vi "Render_AD_Results.vi"(4 "Background Color":u32(colorbox)=16448250, 5 "Rel._Margin":sgl=0.01, 8 "error in":errorcluster, 11 "Anomaly Detection Rresults":T1={"Image"="remote image 000001443E0F18B8", "Ground Truth"="remote image 000001443E0F3018", "Predicted Heat Map"="remote image 000001443E0F25C8", "Predicted Mask"="remote image 000001443E0F1808", "Segmentation"="remote image 000001443E0F2E08"}) -> (0 "error out":errorcluster, 3 "Anomaly Detection Result":T2(plugin-control))   [LabVIEW 2020]
uses:
  Controls/Anomaly_Detection_Results_Imgs.ctl
  <vilib>/vision/NI_Vision_Development_Module.lvlib
panel:
  out "Font Size 2":i16
  in  "Desired Font (Application)":T3(ring)
  in  "[User-specified Font].Font Name":string="system font"
  in  "Horizontal Alignment":i16(ring)=1 items=["Left", "Center", "Right"]
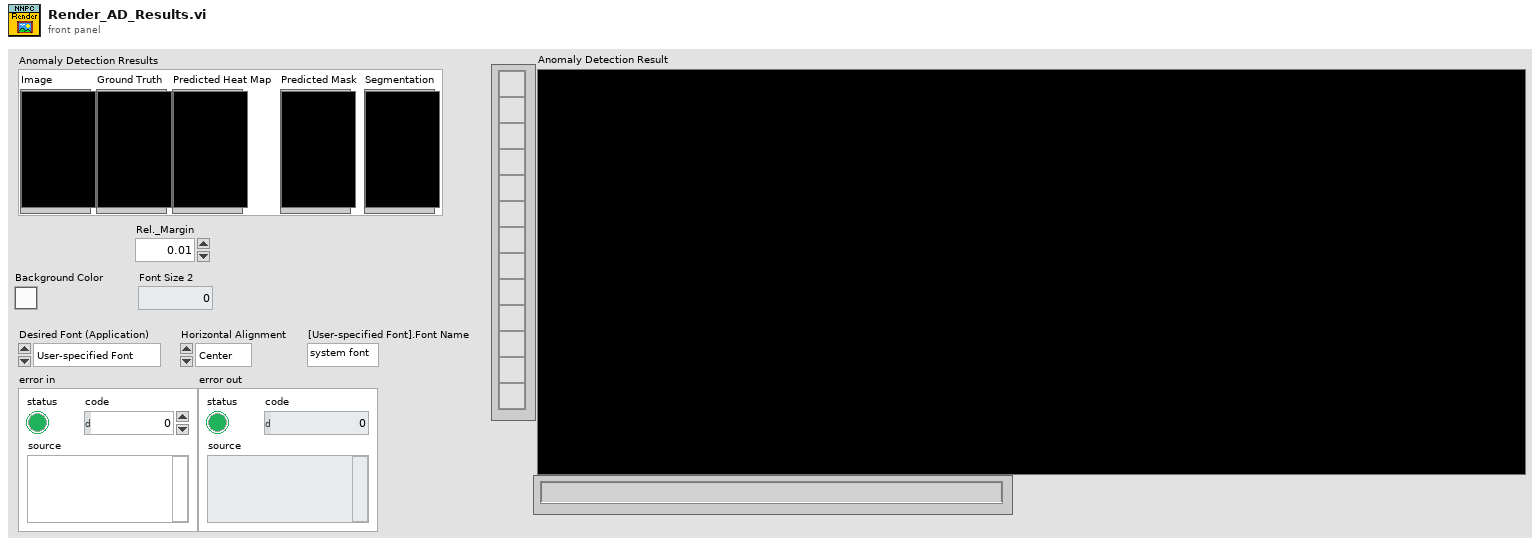
[diagram p1: front panel]
types:
  T1 = typedef "Anomaly_Detection_Results_Imgs.ctl" = cluster{"Image":T2, "Ground Truth":T2, "Predicted Heat Map":T2, "Predicted Mask":T2, "Segmentation":T2}
  T2 = typedef "IMAQ Image.ctl" = refnum<image>
  T3 = enum16{"User-specified Font", "Application Font", "System Font", "Dialog Font"}
  T4 = cluster{"Desired Font (Application)":enum16{"User-specified Font", "Application Font", "System Font", "Dialog Font"}, "[User-specified Font]":cluster{"Font Name":string, "Size":i16, "Strikeout?":bool, "Italic?":bool, "Underline?":bool, "Outline?":bool, "Shadow?":bool, "Bold?":bool, "Rotation Angle":dbl}, "Horizontal Alignment":i16, "Vertical Alignment":i16}
  T5 = typedef "Image Type" = u32
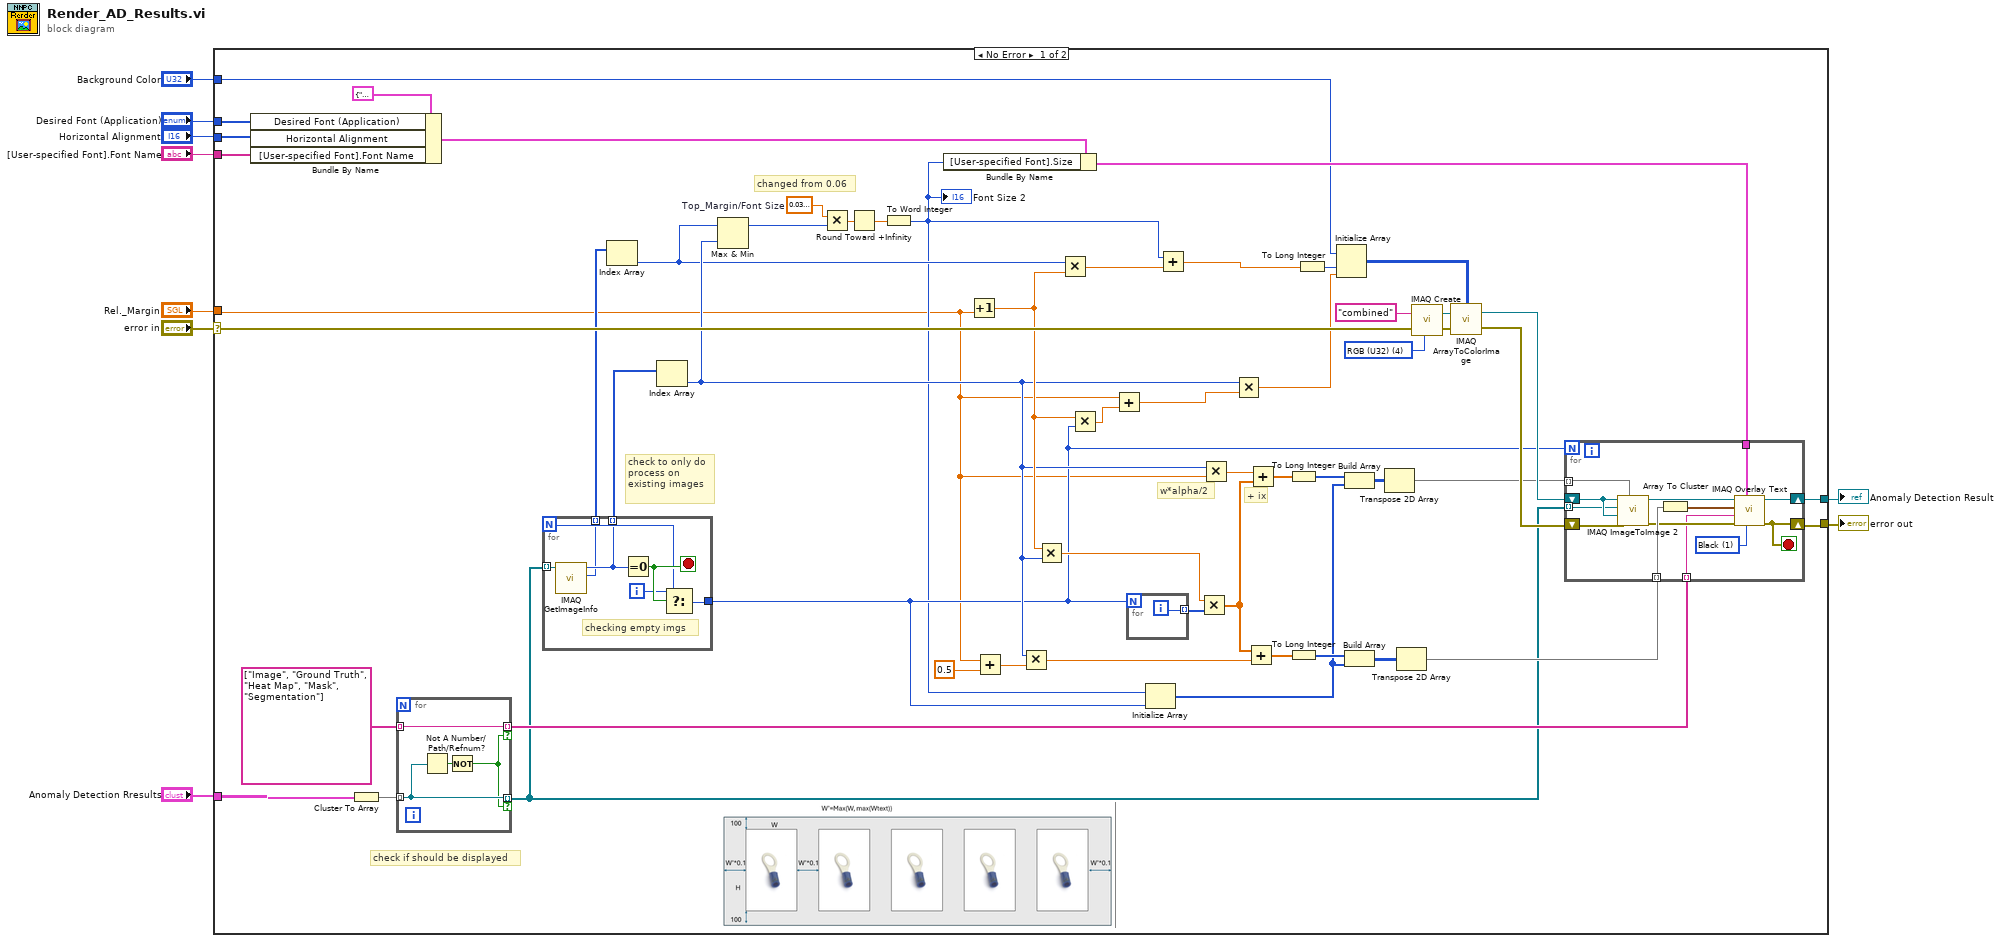
[diagram p0: block diagram]
diagram:
  n1 = case shown="No Error" "error in" {
    selector: "error in" -> [w61 w91]
    tunnel: "Horizontal Alignment" -> [w65 _]
    tunnel: "[User-specified Font].Font Name" -> [w64 _]
    tunnel: "Desired Font (Application)" -> [w63 _]
    tunnel: [w59 w91] -> w3
    tunnel: [w60 _] -> w4
    tunnel: "Anomaly Detection Rresults" -> [w62 _]
    tunnel: "Rel._Margin" -> [w11 _]
    tunnel: "Background Color" -> [w10 _]
    frame No Error {
      w23 = sgl 0.04  # Top_Margin/Font Size
      w58 = T5 4 items=["Grayscale (U8)", "Grayscale (I16)", "Grayscale (SGL)", "Complex (CSG)", "RGB (U32)", "HSL (U32)", "RGB (U64)", "Grayscale (U16)"] ("Image Type")
      # "changed from 0.06"
      # "check if should be displayed"
      # "+ ix"
      # "w*alpha/2"
      # "check to only do process on existing images"
      n2 = Bundle By Name(cluster=T4 {"Desired Font (Application)"=enum."Application Font", "[User-specified Font]"={"Font Name"="", "Size"=12, "Strikeout?"=FALSE, "Italic?"=FALSE, "Underline?"=FALSE, "Outline?"=FALSE, "Shadow?"=FALSE, "Bold?"=FALSE, "Rotation Angle"=0.0}, "Horizontal Alignment"=0, "Vertical Alignment"=0} ("Font, Size & Style"), "Desired Font (Application)"=w63, "Horizontal Alignment"=w65, "[User-specified Font].Font Name"=w64) -> (w39:T4)
      n3 = Cluster To Array(cluster=w62) -> (array=w24:T2[])
      n4 = for {
        tunnel: w24 -> [w89] mode=indexing
        tunnel: string[] ["Image", "Ground Truth", "Heat Map", "Mask", "Segmentation"] ("String") -> [w90] mode=indexing
        tunnel: [w90] -> w25 mode=indexing if=w87
        tunnel: [w89] -> w20 mode=indexing if=w87
        n5 = Not A Number/Path/Refnum?(number/path/refnum=w89) -> (NaN/Path/Refnum?=w88:bool)
        n6 = Not(x=w88) -> (.not. x?=w87:bool)
      }
      n7 = for {
        N -> [w82]
        tunnel: w20 -> [w86] mode=indexing
        tunnel: [w85] -> w14
        tunnel: [w81] -> w36 mode=indexing
        tunnel: [w80] -> w35 mode=indexing
        i -> [w83]
        stop <- w84 stop-if-true
        # "checking empty imgs"
        n8 = call "IMAQ GetImageInfo"("Image"=w86) -> ("Y Resolution"=w80:i32, "X Resolution"=w81:i32)  [unwired: 3 in, 6 out]
        n9 = Equal To 0?(x=w81) -> (x = 0?=w84:bool)
        n10 = Select(t=w83, s=w84, f=w82) -> (s? t:f=w85:i32)
      }
      n11 = Index Array(array=w35) -> (element=w15:i32)  [unwired: 1 in]
      n12 = Index Array(array=w36) -> (element=w16:i32)  [unwired: 1 in]
      n13 = Max & Min(x=w15, y=w16) -> (max(x,y)=w19:i32)  [unwired: 1 out]
      n14 = Multiply(x=w23, y=w19) -> (x*y=w40:sgl)
      n15 = Round Toward +Infinity(x=w40) -> (ceil(x): smallest int >= x=w37:sgl)
      n16 = To Word Integer(number=w37) -> (16bit integer=w13:i16)
      "Font Size 2" <- w13
      n17 = Bundle By Name(cluster=w39, "[User-specified Font].Size"=w13) -> (w38:T4)
      n18 = Increment(x=w11) -> (x+1=w17:sgl)
      n19 = Add(x=w11, y=sgl 0.5) -> (x+y=w45:sgl)
      n20 = Multiply(x=w16, y=w45) -> (x*y=w44:sgl)
      n21 = Multiply(x=w17, y=w16) -> (x*y=w30:sgl)
      n22 = Multiply(x=w15, y=w17) -> (x*y=w28:sgl)
      n23 = Multiply(x=w17, y=w14) -> (x*y=w22:sgl)
      n24 = Add(x=w11, y=w22) -> (x+y=w21:sgl)
      n25 = for {
        N: w14 -> [_]
        tunnel: [w79] -> w48 mode=indexing
        i -> [w79]
      }
      n26 = Initialize Array(w13, w14) -> (w12:i16[])
      n27 = Add(x=w13, y=w28) -> (x+y=w18:sgl)
      n28 = Multiply(x=w30, y=w48) -> (x*y=w34:sgl[])
      n29 = Multiply(x=w16, y=w11) -> (x*y=w31:sgl)
      n30 = Multiply(x=w16, y=w21) -> (x*y=w29:sgl)
      n31 = Add(x=w34, y=w44) -> (x+y=w47:sgl[])
      n32 = Add(x=w31, y=w34) -> (x+y=w27:sgl[])
      n33 = To Long Integer(number=w27) -> (32bit integer=w42:i32[])
      n34 = To Long Integer(number=w47) -> (32bit integer=w43:i32[])
      n35 = To Long Integer(number=w18) -> (32bit integer=w41:i32)
      n36 = Initialize Array(w10, w41, w29) -> (w56:u32[][])
      n37 = Build Array(w42, w12) -> (w53:i32[][])
      n38 = Build Array(w43, w12) -> (w52:i32[][])
      n39 = Transpose 2D Array(2D array=w53) -> (transposed array=w32:i32[][])
      n40 = Transpose 2D Array(2D array=w52) -> (transposed array=w33:i32[][])
      n41 = call "IMAQ Create"("Image Name"="combined", "Image Type"=w58, "error in (no error)"=w61) -> ("New Image"=w55:T2, "error out"=w50:errorcluster)  [unwired: 2 in]
      n42 = call "IMAQ ArrayToColorImage"("Image Pixels (U32)"=w56, "Image"=w55, "error in (no error)"=w50) -> ("Image Out"=w54:T2, "error out"=w49:errorcluster)  [unwired: 2 in]
      n43 = for {
        N: w14 -> [_]
        tunnel: w20 -> [w67] mode=indexing
        shift-right: [w76] -> w60
        shift-left: w54 -> [w78]
        tunnel: w25 -> [w72] mode=indexing
        tunnel: w33 -> [w75] mode=indexing
        tunnel: w38 -> [w74]
        shift-right: [w71] -> w59
        shift-left: w49 -> [w66]
        tunnel: w32 -> [w68] mode=indexing
        stop <- w71 stop-if-true
        w70 = 1 items=["White", "Black", "Inverted", "Black on White", "White on Black"] ("Color")
        n44 = call "IMAQ ImageToImage 2"("Offset Left/Top"=w68, "error in (no error)"=w66, "Image Dst"=w78, "Image Src (Small)"=w67, "Image Src (Large)"=w78) -> ("error out"=w73:errorcluster, "Image Dst Out"=w77:T2)  [unwired: 5 in]
        n45 = Array To Cluster(array=w75) -> (cluster=w69:cluster{"[0]":i32, "[1]":i32})
        n46 = call "IMAQ Overlay Text"("Text Color (black)"=w70, "Font, Size & Style"=w74, "error in (no error)"=w73, "String"=w72, "Origin"=w69, "Image"=w77) -> ("error out"=w71:errorcluster, "Image Out"=w76:T2)  [unwired: 4 in]
      }
    }
    frame Error {
    }
  }
  "Anomaly Detection Result" <- w4
  "error out" <- w3
